vi "GetClassTemplates.vi"(0 "ClassWriterNative in":refnum<class "ClassWriterNative.lvclass">, 1 "DerivedFromThisClass(if any)":refnum<vi>, 5 "error in (no error)":errorcluster) -> (14 "ClassWriterNative out":refnum<class "ClassWriterNative.lvclass">, 15 "Templates(Matching Connector Pane Settings)":T1[](array[typedef]), 16 "AllTemplateNames(FolderNames)":string[](array[string]), 19 "error out":errorcluster)   [LabVIEW 2020, in "ClassWriterNative.lvclass"]
uses:
  <resource>/Framework/Providers/Open_GDS/ClassProviders/Provider_LvNativeClass/ClassWriterNative_class/ClassWriterNative.lvclass
  <resource>/Framework/Providers/Open_GDS/ClassProviders/Provider_BaseClassInterface/ClassTemplateType.ctl
  <resource>/Framework/Providers/Open_GDS/ClassProviders/Common/ScriptingFunctions/Scripting_ConnectorPanePatternType.ctl
  <resource>/Framework/Providers/Open_GDS/ClassProviders/Provider_LvNativeClass/ClassWriterNative_class/ClassWriterNative.lvclass/ClassWriterNative.ctl
  <resource>/Framework/Providers/Open_GDS/ClassProviders/Provider_BaseClassInterface/ClassWriter_class/ClassWriter.lvclass
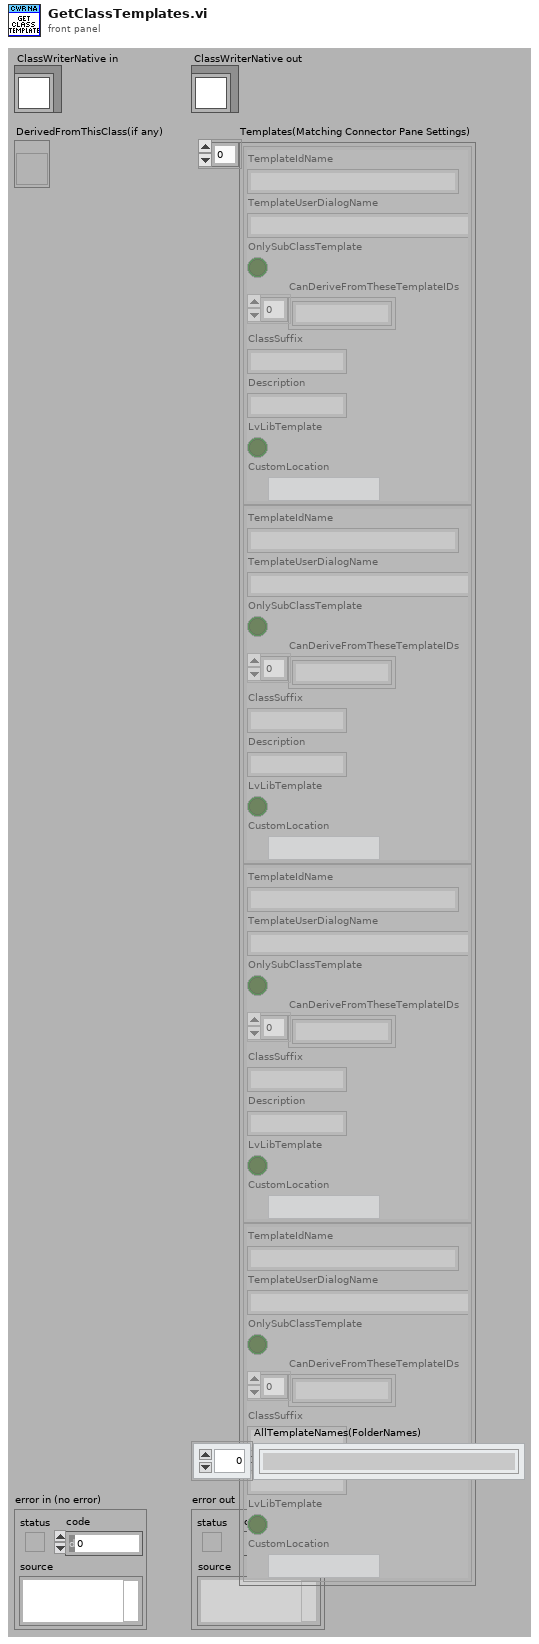
[diagram p1: front panel]
types:
  T1 = typedef "ClassWriter.lvclass/ClassTemplateType.ctl" = cluster{"TemplateIdName":string, "TemplateUserDialogName":string, "OnlySubClassTemplate":bool, "CanDeriveFromTheseTemplateIDs":string[], "ClassSuffix":string, "Description":string, "LvLibTemplate":bool, "CustomLocation":path}
  T2 = typedef "Scripting_ConnectorPanePatternType.ctl" = u16
  T3 = typedef "GDSLvCLass_ClassSettingsType.ctl" = cluster{"ClassProviderName":string, "ClassTemplateUsed":string, "ClassTemplateVersion":string, "ClassDescription":string, "PlugIns":T4[], "ConnectorPanePattern":string}
  T4 = typedef "GDSLvClass_PlugIn.ctl" = cluster{"Type":T5, "ID":string, "Version":string, "Path":path, "Name":string, "Data":variant}
  T5 = typedef "GDSLvClass_PlugInTypes.ctl" = enum16{"DesignPattern", "MethodTypes"}
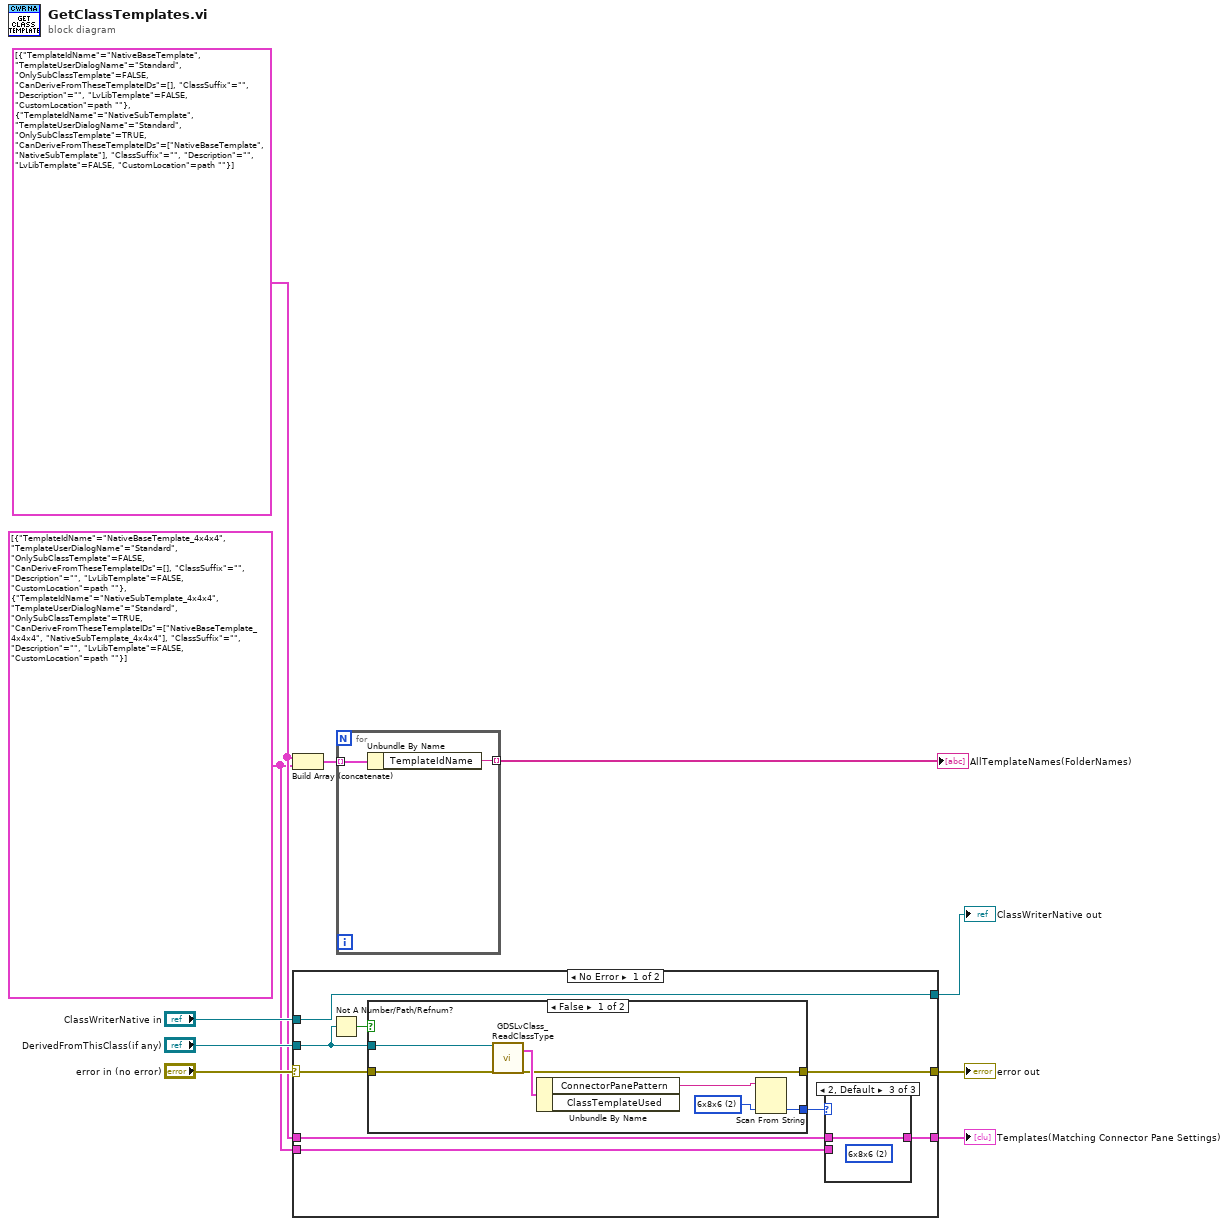
[diagram p0: block diagram]
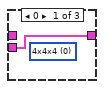
[diagram p2: hidden frame]
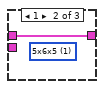
[diagram p3: hidden frame]
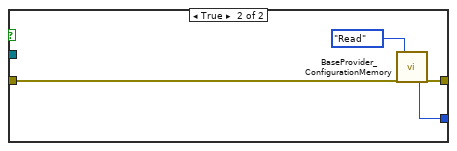
[diagram p4: hidden frame]
diagram:
  w3 = T1[] [{"TemplateIdName"="NativeBaseTemplate_4x4x4", "TemplateUserDialogName"="Standard", "OnlySubClassTemplate"=FALSE, "CanDeriveFromTheseTemplateIDs"=[], "ClassSuffix"="", "Description"="", "LvLibTemplate"=FALSE, "CustomLocation"=path ""}, {"TemplateIdName"="NativeSubTemplate_4x4x4", "TemplateUserDialogName"="Standard", "OnlySubClassTemplate"=TRUE, "CanDeriveFromTheseTemplateIDs"=["NativeBaseTemplate_4x4x4", "NativeSubTemplate_4x4x4"], "ClassSuffix"="", "Description"="", "LvLibTemplate"=FALSE, "CustomLocation"=path ""}] ("TemplateIdNames")
  w4 = T1[] [{"TemplateIdName"="NativeBaseTemplate", "TemplateUserDialogName"="Standard", "OnlySubClassTemplate"=FALSE, "CanDeriveFromTheseTemplateIDs"=[], "ClassSuffix"="", "Description"="", "LvLibTemplate"=FALSE, "CustomLocation"=path ""}, {"TemplateIdName"="NativeSubTemplate", "TemplateUserDialogName"="Standard", "OnlySubClassTemplate"=TRUE, "CanDeriveFromTheseTemplateIDs"=["NativeBaseTemplate", "NativeSubTemplate"], "ClassSuffix"="", "Description"="", "LvLibTemplate"=FALSE, "CustomLocation"=path ""}] ("TemplateIdNames")
  n1 = Build Array (concatenate)(w4, w3) -> (w2:T1[])
  n2 = case shown="No Error" "error in (no error)" {
    selector: "error in (no error)" -> [w15 w35]
    tunnel: [w14 w35] -> w9
    tunnel: [w19 w34] -> w7
    tunnel: "ClassWriterNative in" -> [w19 w34]
    tunnel: [w18 _] -> w5
    tunnel: "DerivedFromThisClass(if any)" -> [w16 _]
    tunnel: w4 -> [w12 _]
    tunnel: w3 -> [w11 _]
    frame No Error {
      n3 = Not A Number/Path/Refnum?(number/path/refnum=w16) -> (NaN/Path/Refnum?=w17:bool)
      n4 = case shown="False" w17 {
        tunnel: w15 -> [w26 w32]
        tunnel: w16 -> [w25 _]
        tunnel: [w24 w31] -> w14
        tunnel: [w23 w30] -> w13
        frame False {
          w27 = T2 2 items=["4x4x4", "5x6x5", "6x8x6"] ("Pattern")
          n5 = call <resource>:"GDSLvClass_ReadClassType.vi"("Class Refnum In"=w25, "error in (no error)"=w26) -> ("ClassSettings"=w29:T3, "error out"=w24:errorcluster)  [unwired: 15 in, 1 out]
          n6 = Unbundle By Name(w29) -> ("ConnectorPanePattern"=w28:string)  [unwired: 1 out]
          n7 = Scan From String(input string=w28, default 1=w27) -> (output 1=w23:T2)  [unwired: 3 in, 3 out]
        }
        frame True {
          n8 = call <resource>:"BaseProvider_ConfigurationMemory.vi"("error in (no error)"=w32, "Action"=enum16{"Read", "Load", "Save"}."Read") -> ("PatternOut"=w30:T2, "error out"=w31:errorcluster)  [unwired: 11 in, 5 out]
        }
      }
      n9 = case shown="2, Default" w13 {
        tunnel: [w20 w21 w22] -> w18
        tunnel: w12 -> [_ w21 w22]
        tunnel: w11 -> [w20 _ _]
        frame 0 {
          (unwired) T2 0 items=["4x4x4", "5x6x5", "6x8x6"] ("Pattern")
        }
        frame 1 {
          (unwired) T2 1 items=["4x4x4", "5x6x5", "6x8x6"] ("Pattern")
        }
        frame 2, Default {
          (unwired) T2 2 items=["4x4x4", "5x6x5", "6x8x6"] ("Pattern")
        }
      }
    }
    frame Error {
    }
  }
  "error out" <- w9
  "ClassWriterNative out" <- w7
  "Templates(Matching Connector Pane Settings)" <- w5
  n10 = for {
    tunnel: w2 -> [w37] mode=indexing
    tunnel: [w36] -> w1 mode=indexing
    n11 = Unbundle By Name(w37) -> ("TemplateIdName"=w36:string)
  }
  "AllTemplateNames(FolderNames)" <- w1
